vi "Native_GetForTunnels.vi"() -> ()   [LabVIEW 2024]
panel:
  out "error out":errorcluster caption="错误输出"
  out "tunnel_ids":u32[](array[numeric])
  in  "tunnel_ids type":u32
  in  "for_id":u32
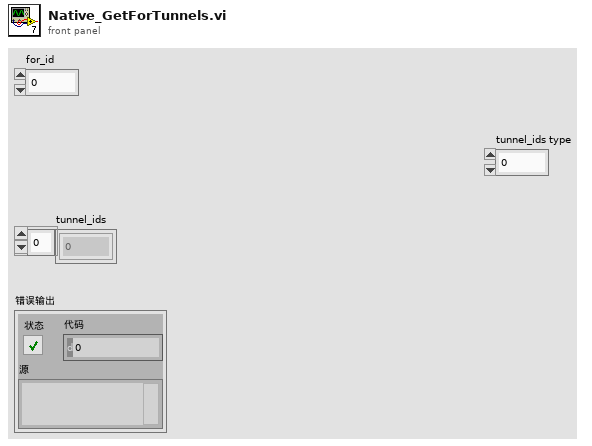
[diagram p1: front panel]
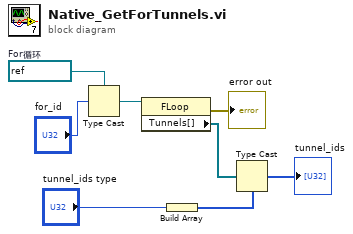
[diagram p0: block diagram]
diagram:
  w7 = refnum<vi> refnum  # For循环
  n1 = Type Cast ("强制类型转换")(type=w7, x="for_id") -> (*(type *) &x=w6:refnum<vi>)
  n2 = property on="属性节点" class="FLoop"(reference=w6) -> (error out=→"error out":errorcluster, "Tunnels[]"=w5:refnum<vi>[])  [unwired: 1 in, 1 out]
  n3 = Build Array ("创建数组")("tunnel_ids type") -> (w3:u32[])
  n4 = Type Cast ("强制类型转换")(type=w3, x=w5) -> (*(type *) &x=→"tunnel_ids":u32[])
